vi "Torque_Feedback.vi"(8 "error in (no error)":errorcluster, 11 "Motor in":refnum<class "Motor.lvclass">) -> (0 "error out":errorcluster, 2 "Actual Torque":dbl, 3 "Motor out":refnum<class "Motor.lvclass">)   [LabVIEW 2021, in "Motor.lvclass"]
uses:
  Motor.lvclass
  Motor.lvclass/Motor.ctl
  AnalogInput/AnalogInput.lvclass
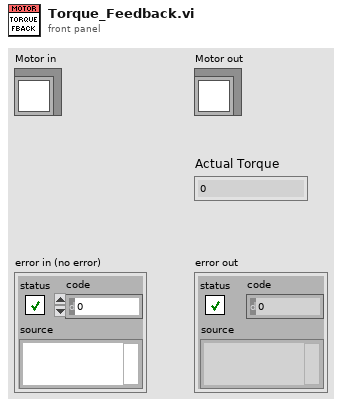
[diagram p1: front panel]
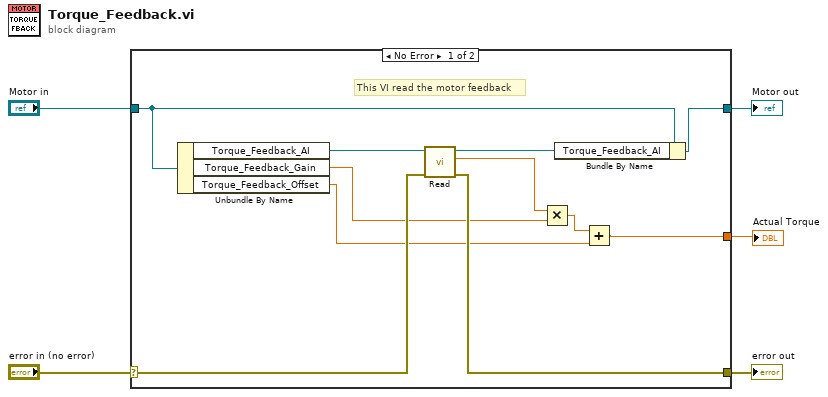
[diagram p0: block diagram]
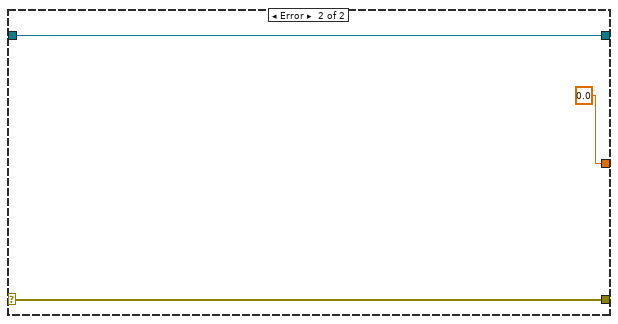
[diagram p2: hidden frame]
diagram:
  n1 = case shown="No Error" "error in (no error)" {
    selector: "error in (no error)" -> [w16 w19]
    tunnel: [w14 w19] -> w4
    tunnel: [w11 w18] -> w2
    tunnel: "Motor in" -> [w13 w18]
    tunnel: [w8 0.0 ("Data Out")] -> w1
    frame No Error {
      # "This VI read the motor feedback"
      n2 = Unbundle By Name(w13) -> ("Torque_Feedback_AI"=w15:refnum<class "AnalogInput.lvclass">, "Torque_Feedback_Gain"=w7:dbl, "Torque_Feedback_Offset"=w6:dbl)
      n3 = call-dynamic "Read.vi"("error in (no error)"=w16, "AnalogInput in"=w15) -> ("error out"=w14:errorcluster, "Data Out"=w10:dbl, "AnalogInput out"=w12:refnum<class "AnalogInput.lvclass">)  [unwired: 7 in]
      n4 = Multiply(x=w10, y=w7) -> (x*y=w9:dbl)
      n5 = Bundle By Name(cluster=w13, "Torque_Feedback_AI"=w12) -> (w11:refnum<class "Motor.lvclass">)
      n6 = Add(x=w9, y=w6) -> (x+y=w8:dbl)
    }
    frame Error {
    }
  }
  "error out" <- w4
  "Motor out" <- w2
  "Actual Torque" <- w1
